vi "LabVIEW.FGV.Creat_Result.vi"(7 "Command":enum16{"write", "read", "clear"}(ring), 8 "error in (no error)":errorcluster caption="Fehler (Eingang, kein Fehler)", 10 "Passed?":bool, 11 "Result_Cluster":T1) -> (0 "error out":errorcluster caption="Fehler (Ausgang)", 3 "Angehängtes Array":string[][](array[string]))   [LabVIEW 2019]
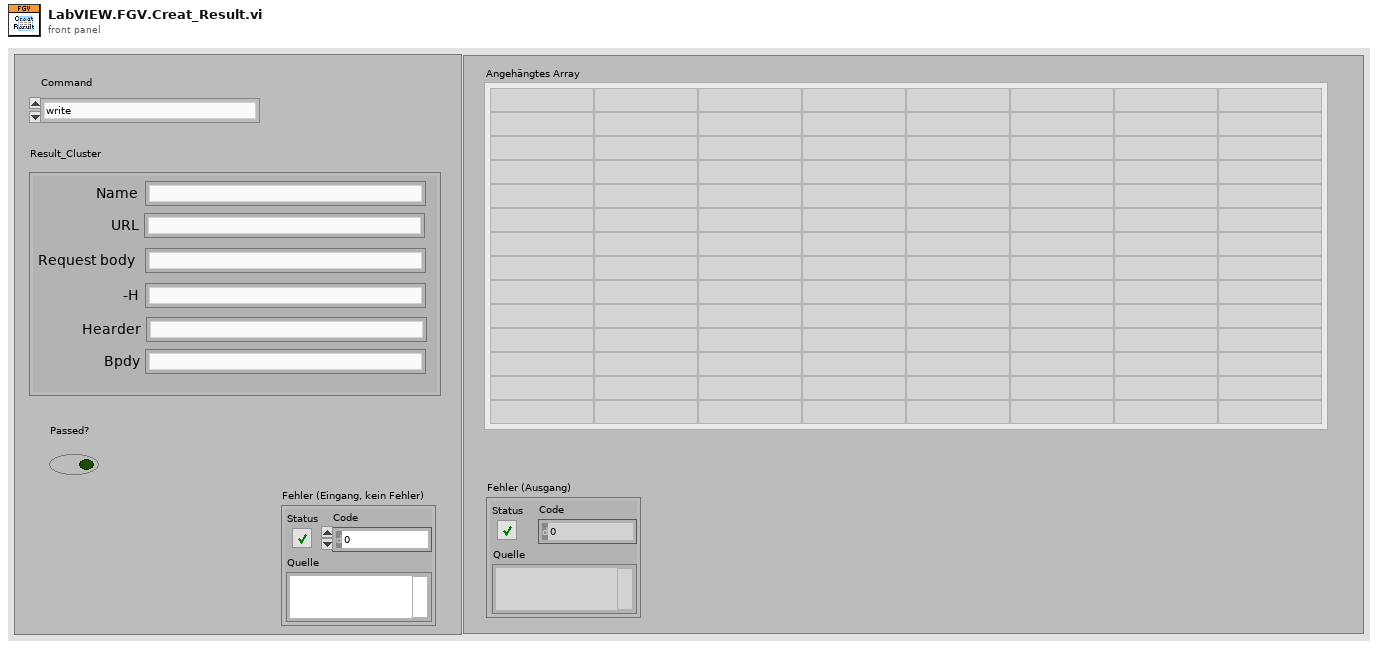
[diagram p1: front panel]
types:
  T1 = cluster{"Name":string, "URL":string, "Request body":string, "-H":string, "Hearder":string, "Bpdy":string}
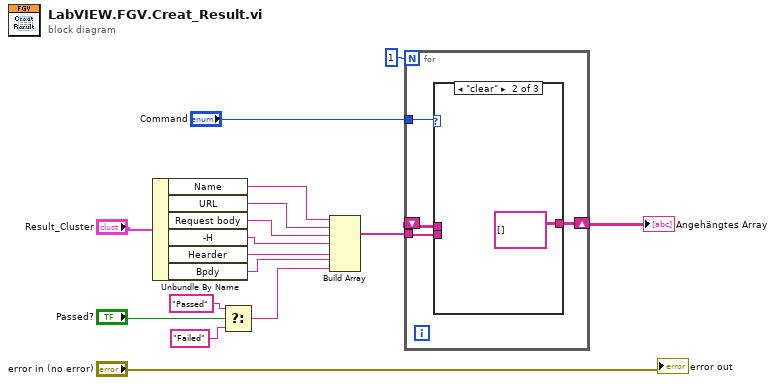
[diagram p0: block diagram]
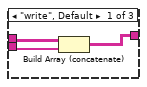
[diagram p2: hidden frame]
diagram:
  n1 = Unbundle By Name("Result_Cluster") -> ("Name"=w12:string, "URL"=w11:string, "Request body"=w10:string, "-H"=w9:string, "Hearder"=w8:string, "Bpdy"=w7:string)
  n2 = Select(t="Passed", s="Passed?", f="Failed") -> (s? t:f=w6:string)
  n3 = Build Array(w12, w11, w10, w9, w8, w7, w6) -> (w5:string[])
  n4 = for {
    N: 1 -> [_]
    tunnel: w5 -> [w20]
    shift-right: [w19] -> w4
    shift-left: _ -> [w18]
    tunnel: "Command" -> [w17]
    n5 = case shown="\"clear\"" w17 {
      tunnel: w20 -> [w21 _ _]
      tunnel: [w23 string[][] [] w25] -> w19
      tunnel: w18 -> [w22 _ w25]
      frame "write", Default {
        n6 = Build Array (concatenate)(w22, w21) -> (w23:string[][])
      }
      frame "clear" {
      }
      frame "read" {
      }
    }
  }
  "Angehängtes Array" <- w4
  "error out" <- "error in (no error)"
